vi "MDPtr DAQ Example.vi"() -> ()   [LabVIEW 2017]
uses:
  MDPtr TypeDef/MDPtr DataFrame-Common.ctl
  <vilib>/Utility/Data Type/Type Definitions/Data Type.ctl
  MDPtr TypeDef/MDPtr.ctl
  4b70eac3-4565-41a8-8678-ce1595016193.vi
  8e4e57da-1b82-406e-8431-dbf41ec60265.vi
  d8984c18-04cb-4ba4-ae9b-6c5b3b1c3ef6.vi
  9cd2cd57-26eb-46a0-897a-d177a379a7ae.vi
  54395307-d518-4202-990a-94b812b105bc.vi
  _MDPtrMgr/MallocMethod/MallocMethod-FIXED-PRESIZE.vi
  <vilib>/Utility/Data Type/Get Type Information.vi
  _Support/_MDPtr Validate DataFrame Type.vi
  _Support/_MDPtr Unpack Memory.vi
  _Support/_MDPtr DecrementCount.vi
  _Support/_MDPtr Pack Memory.vi
  MDPtr.lvlib
  <vilib>/measure/NI_MABase.lvlib
  _MDPtrMgr/MDPtrMgr.lvclass
  <vilib>/Utility/Data Type/NI_Data Type.lvlib
panel:
  out "Sine":waveform(dbl)(graph)
  out "Square":waveform(dbl)(graph)
  in  "Logging?":bool
  out "File Logging?":bool
  in  "file path":path=path "D:/MDPtr.tdms"
  in  "stop":bool
  in  "CacheSize(-1 to Free All caches)":i32=-1
  in  "clean caches":bool
  out "Information":T1
  out "time esliped(s)":dbl
  in  "milliseconds to wait 2":u32=1
  out "Cache Names":string[](array[string])
  in  "Fs":dbl=1000.0 format="%#_13g"
  out "# free MDPtrs in caches":i32
  out "# MDPtrs allocated":i32
  out "# caches":i32
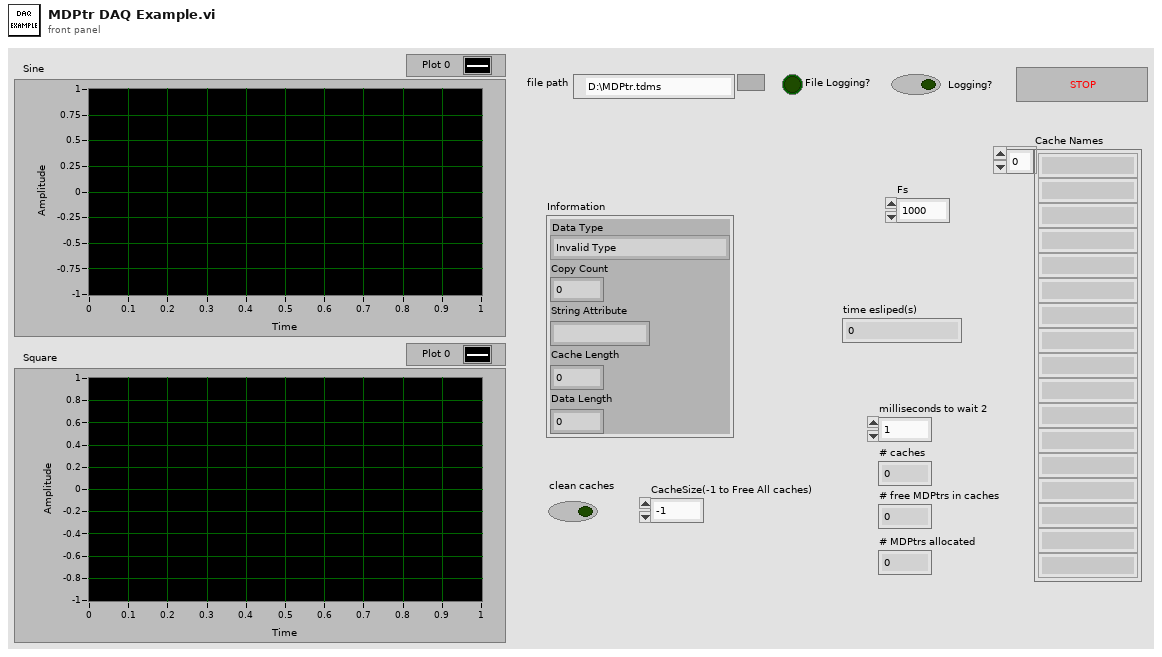
[diagram p1: front panel]
types:
  T1 = typedef "MDPtr.lvlib/MDPtr DataFrame-Common.ctl" = cluster{"Data Type":T2, "Copy Count":i32, "String Attribute":string, "Cache Length":i32, "Data Length":i32}
  T2 = typedef "NI_Data Type.lvlib/Data Type.ctl" = enum8{"Invalid Type", "Void", "I8", "I16", "I32", "I64", "U8", "U16", "U32", "U64", "Single Float", "Double Float", "Extended Float", "Single Complex", "Double Complex", "Extended Complex", "Enum U8", "Enum U16", "Enum U32", "Enum U64", "Single Float With Unit", "Double Float With Unit", "Extended Float With Unit", "Single Complex with Unit", "Double Complex with Unit", "Extended Complex with Unit", "Boolean", "String", "Path", "Picture", "Tag", "Array", "Cluster", "Variant", "LV Variant", "Waveform", "Timestamp", "Digital Waveform", "Digital Data", "ExpressData", "Refnum", "External Data", "VI", "Poly VI", "LabVIEW Class Instance", "Fixed Point"}
  T3 = enum16{"open", "open or create", "create or replace", "create", "open (read-only)"}
  T4 = typedef "MDPtr.lvlib/MDPtr.ctl" = refnum<k1>
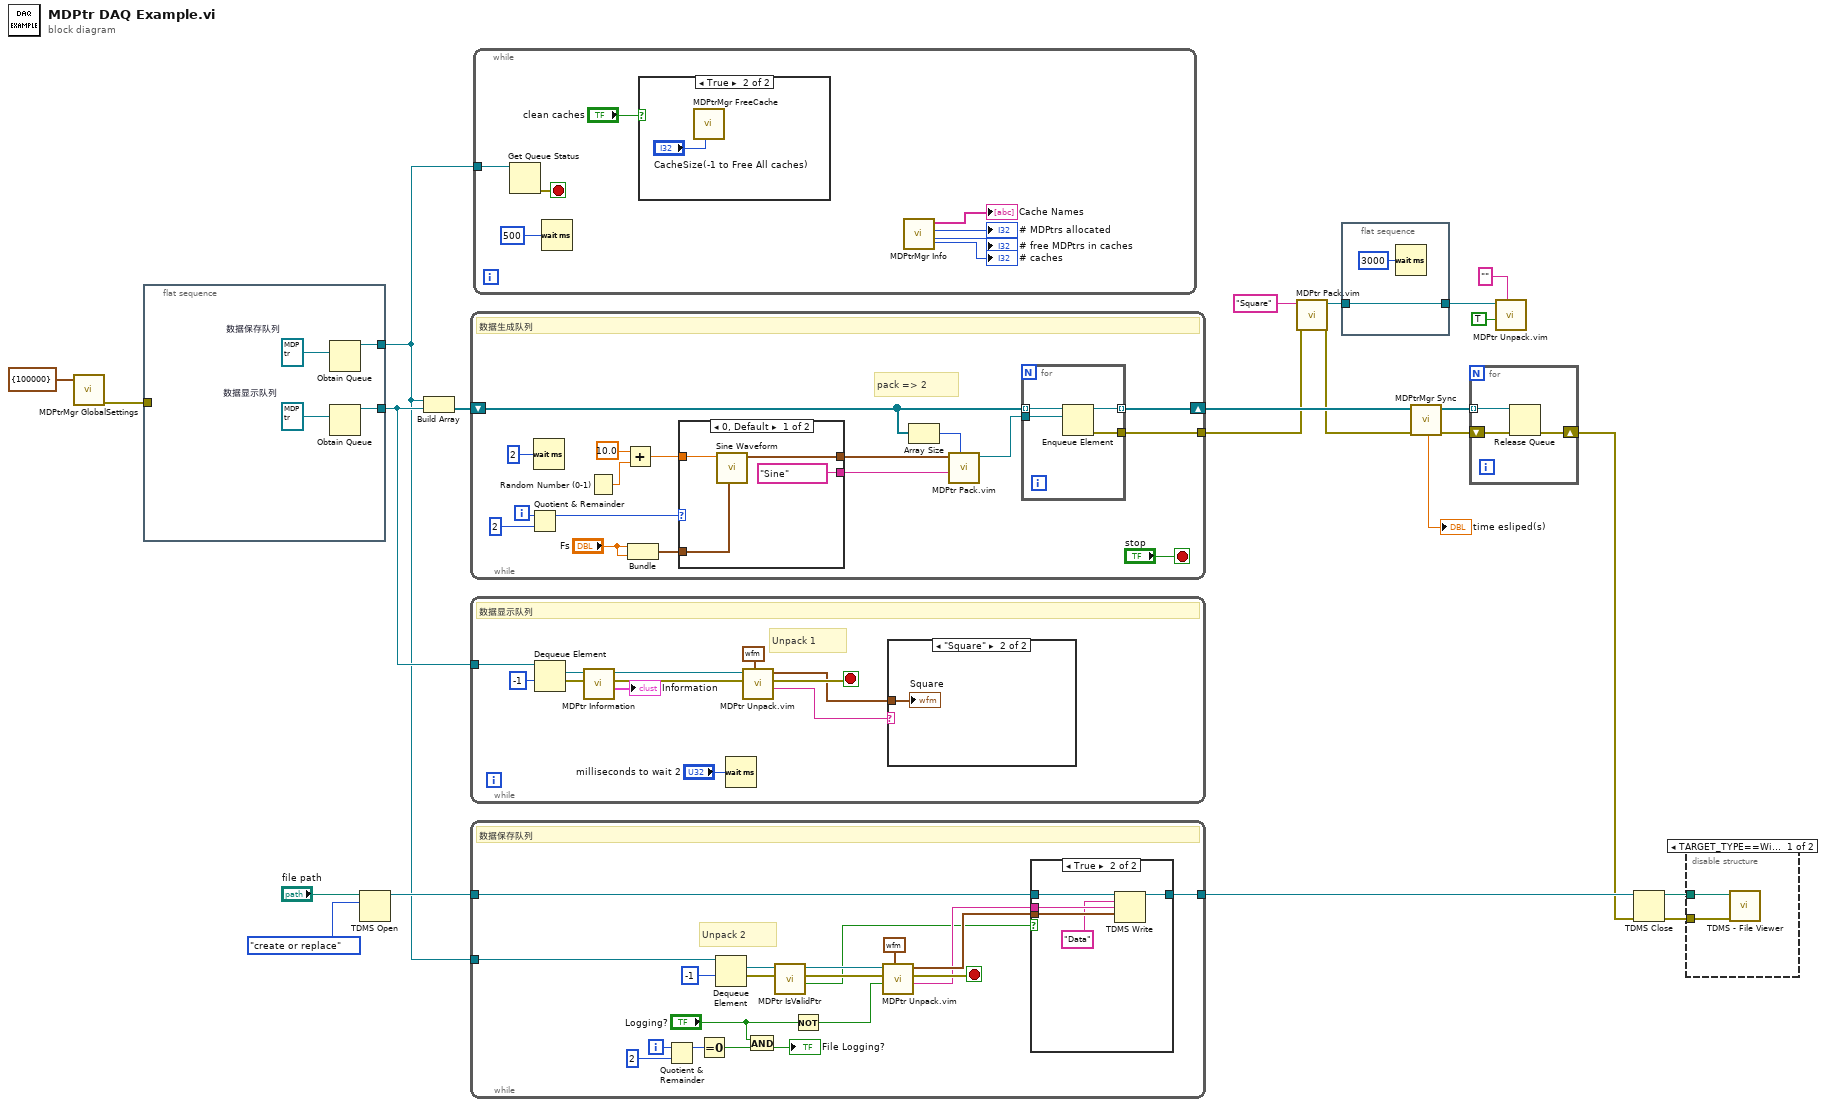
[diagram p0: block diagram]
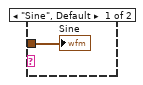
[diagram p5: hidden frame]
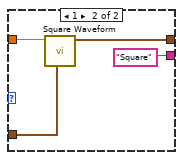
[diagram p6: hidden frame]
diagram:
  n1 = call-poly "MDPtrMgr GlobalSettings.vi"("FixedPreSize"=cluster{"PreCacheSize":i32} {"PreCacheSize"=100000}) -> ("error out"=w14:errorcluster)  [unwired: 10 in]
  n2 = flat-sequence {
    tunnel: [w24] -> w21
    tunnel: [w23] -> w2
    tunnel: w14 -> [_]
    frame #0 {
      n3 = Obtain Queue "数据保存队列"(element data type=T4 refnum ("MDPtr")) -> (queue out=w23:refnum<queue>)  [unwired: 4 in, 2 out]
      n4 = Obtain Queue "数据显示队列"(element data type=T4 refnum ("MDPtr")) -> (queue out=w24:refnum<queue>)  [unwired: 4 in, 2 out]
    }
  }
  n5 = TDMS Open(10:T3."create or replace" ("operation (0:open)"), 11:"file path") -> (3:w19:refnum<k34>)  [unwired: 5 in, 1 out]
  n6 = Build Array(w2, w21) -> (w3:refnum<queue>[])
  n7 = while {
    shift-right: [w43] -> w17
    shift-left: w3 -> [w29]
    tunnel: [w30] -> w5
    i -> [w41]
    stop <- "stop" stop-if-true
    # "pack => 2"
    # "数据生成队列"
    n8 = Quotient & Remainder(x=w41, y=2) -> (x-y*floor(x/y)=w39:i32)  [unwired: 1 out]
    n9 = Wait (ms)(milliseconds to wait=u32 2) -> ()  [unwired: 1 out]
    n10 = Random Number (0-1)() -> (number: 0 to 1=w35:dbl)
    n11 = Add(x=10.0 ("frequency"), y=w35) -> (x+y=w34:dbl)
    n12 = Bundle("Fs"="Fs", "Fs"="Fs") -> (w31:cluster{"Fs":dbl, "Fs":dbl})  [unwired: 1 in]
    n13 = case shown="0, Default" w39 {
      tunnel: [w51 w55] -> w33
      tunnel: ["Sine" ("String Attribute") "Square" ("String Attribute")] -> w38
      tunnel: w34 -> [w49 w53]
      tunnel: w31 -> [w48 w52]
      frame 0, Default {
        n14 = call <vilib>:"Sine Waveform.vi"("sampling info"=w48, "frequency"=w49) -> ("signal out"=w51:waveform(dbl))  [unwired: 8 in, 1 out]
      }
      frame 1 {
        n15 = call <vilib>:"Square Waveform.vi"("sampling info"=w52, "frequency"=w53) -> ("signal out"=w55:waveform(dbl))  [unwired: 8 in, 1 out]
      }
    }
    n16 = Array Size(array=w29) -> (size(s)=w28:i32)
    n17 = call "MDPtr Pack.vim"("Copies Count(1)"=w28, "String Attribute"=w38, "Data"=w33) -> ("HexStrPtr"=w27:T4)  [unwired: 7 in, 1 out]
    n18 = for {
      tunnel: [w47] -> w43 mode=indexing
      tunnel: [w46] -> w30
      tunnel: w29 -> [w45] mode=indexing
      tunnel: w27 -> [w44]
      n19 = Enqueue Element(queue=w45, element=w44) -> (queue out=w47:refnum<queue>, error out=w46:errorcluster)  [unwired: 2 in, 1 out]
    }
  }
  n20 = while {
    tunnel: w21 -> [w67]
    stop <- w65 stop-if-true
    # "Unpack 1"
    # "数据显示队列"
    n21 = Dequeue Element(queue=w67, timeout in ms (-1)=-1) -> (element=w59:T4, error out=w64:errorcluster)  [unwired: 1 in, 2 out]
    n22 = call "MDPtr Information.vi"("error in (no error)"=w64, "HexStrPtr"=w59) -> ("Information"=→"Information":T1, "error out"=w63:errorcluster, "HexStrPtr (dup)"=w62:T4)  [unwired: 7 in]
    n23 = Wait (ms)(milliseconds to wait="milliseconds to wait 2") -> ()  [unwired: 1 out]
    n24 = call "MDPtr Unpack.vim"("Prototype"=waveform(dbl) {"t0"=timestamp(0 s since 1904-01-01), "dt"=1.0, "Y"=[]} ("Square"), "error in (no error)"=w63, "HexStrPtr"=w62) -> ("String Attribute"=w61:string, "error out"=w65:errorcluster, "Data"=w60:waveform(dbl))  [unwired: 6 in]
    n25 = case shown="\"Square\"" w61 {
      tunnel: w60 -> [w68 w69]
      frame "Sine", Default {
        "Sine" <- w68
      }
      frame "Square" {
        "Square" <- w69
      }
    }
  }
  n26 = while {
    tunnel: w2 -> [w89]
    tunnel: [w84] -> w20
    tunnel: w19 -> [w85]
    i -> [w76]
    stop <- w87 stop-if-true
    # "Unpack 2"
    # "数据保存队列"
    n27 = Quotient & Remainder(x=w76, y=2) -> (x-y*floor(x/y)=w75:i32)  [unwired: 1 out]
    n28 = Equal To 0?(x=w75) -> (x = 0?=w74:bool)
    n29 = Dequeue Element(queue=w89, timeout in ms (-1)=-1) -> (element=w86:T4, error out=w79:errorcluster)  [unwired: 1 in, 2 out]
    n30 = And(x="Logging?", y=w74) -> (x .and. y?=→"File Logging?":bool)
    n31 = call "MDPtr IsValidPtr.vi"("error in (no error)"=w79, "HexStrPtr"=w86) -> ("Valid MDPtr?"=w78:bool, "error out"=w80:errorcluster, "HexStrPtr (dup)"=w81:T4)  [unwired: 6 in]
    n32 = Not(x="Logging?") -> (.not. x?=w70:bool)
    n33 = call "MDPtr Unpack.vim"("Prototype"=waveform(dbl) {"t0"=timestamp(0 s since 1904-01-01), "dt"=1.0, "Y"=[]} ("Square"), "discard?(F)"=w70, "error in (no error)"=w80, "HexStrPtr"=w81) -> ("String Attribute"=w82:string, "error out"=w87:errorcluster, "Data"=w83:waveform(dbl))  [unwired: 5 in]
    n34 = case shown="True" w78 {
      tunnel: w85 -> [w90 w95]
      tunnel: [w90 w94] -> w84
      tunnel: w83 -> [_ w93]
      tunnel: w82 -> [_ w92]
      frame False {
      }
      frame True {
        n35 = TDMS Write(0:w95, 5:"Data" ("group name in (Untitled)"), 7:w92, 9:w93) -> (4:w94:refnum<k34>)  [unwired: 2 in, 3 out]
      }
    }
  }
  n36 = while {
    tunnel: w2 -> [w103]
    stop <- w102 stop-if-true
    n37 = Get Queue Status(queue=w103) -> (error out=w102:errorcluster)  [unwired: 2 in, 7 out]
    n38 = Wait (ms)(milliseconds to wait=u32 500) -> ()  [unwired: 1 out]
    n39 = case shown="True" "clean caches" {
      frame False {
      }
      frame True {
        n40 = call "MDPtrMgr FreeCache.vi"("CacheSize(-1 to Free All caches)"="CacheSize(-1 to Free All caches)") -> ()  [unwired: 10 in, 1 out]
      }
    }
    n41 = call "MDPtrMgr Info.vi"() -> ("# free MDPtrs in caches"=→"# free MDPtrs in caches":i32, "# MDPtrs allocated"=→"# MDPtrs allocated":i32, "Cache Names"=→"Cache Names":string[], "# caches"=→"# caches":i32)  [unwired: 7 in, 1 out]
  }
  n42 = call "MDPtr Pack.vim"("error in (no error)"=w5, "Data"="Square" ("String Attribute")) -> ("error out"=w4:errorcluster, "HexStrPtr"=w9:T4)  [unwired: 8 in]
  n43 = flat-sequence {
    tunnel: w9 -> [w105]
    tunnel: [w105] -> w8
    frame #0 {
      n44 = Wait (ms)(milliseconds to wait=u32 3000) -> ()  [unwired: 1 out]
    }
  }
  n45 = call "MDPtrMgr Sync.vi"("error in (no error)"=w4) -> ("error out"=w16:errorcluster, "time esliped?"=→"time esliped(s)":dbl)  [unwired: 8 in, 1 out]
  n46 = for {
    tunnel: w17 -> [w109] mode=indexing
    shift-right: [w107] -> w1
    shift-left: w16 -> [w108]
    n47 = Release Queue(queue=w109, error in (no error)=w108) -> (error out=w107:errorcluster)  [unwired: 1 in, 2 out]
  }
  n48 = call "MDPtr Unpack.vim"("Prototype"="" ("String Attribute"), "discard?(F)"=TRUE, "HexStrPtr"=w8) -> ()  [unwired: 6 in, 3 out]
  n49 = TDMS Close(8:w1, 11:w20) -> (0:w12:errorcluster, 3:w11:path)
  n50 = disable-structure shown="TARGET_TYPE==Windows" {
    disable-tunnel: w12 -> [w111 _]
    disable-tunnel: w11 -> [w110 _]
    frame condition #0 (active) {
      n51 = call <vilib>:"TDMS - File Viewer.vi"("error in (no error)"=w111, "file path"=w110) -> ()  [unwired: 4 in, 2 out]
    }
    frame condition #1 {
    }
  }
